vi "Read.vi"(8 "error in (no error)":errorcluster, 11 "Modbus_AI in":refnum<class "Modbus_AI.lvclass">) -> (0 "error out":errorcluster, 2 "Data Out":dbl, 3 "Modbus_AI out":refnum<class "Modbus_AI.lvclass">)   [LabVIEW 2021, in "Modbus_AI.lvclass"]
uses:
  Modbus_AI.lvclass
  Modbus_AI.lvclass/Modbus_AI.ctl
  Modbus_Master/Modbus_Master.lvclass
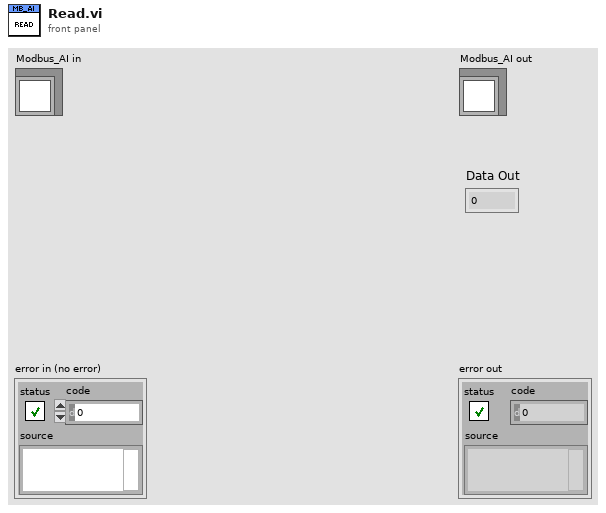
[diagram p1: front panel]
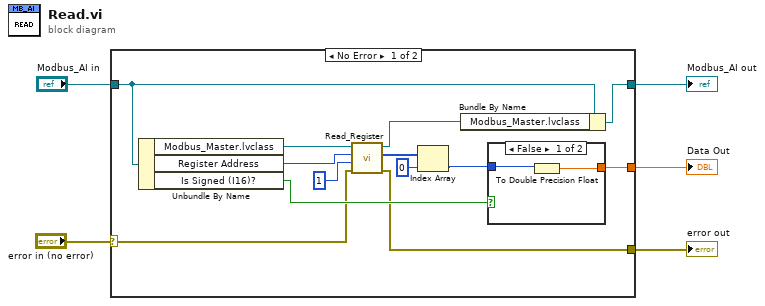
[diagram p0: block diagram]
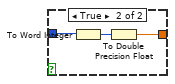
[diagram p2: hidden frame]
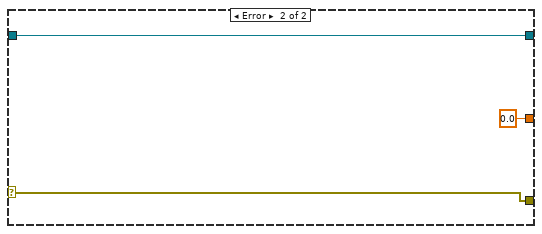
[diagram p3: hidden frame]
diagram:
  n1 = case shown="No Error" "error in (no error)" {
    selector: "error in (no error)" -> [w10 w25]
    tunnel: "Modbus_AI in" -> [w8 w24]
    tunnel: [w11 0.0] -> w3
    tunnel: [w9 w25] -> w2
    tunnel: [w7 w24] -> w1
    frame No Error {
      n2 = Unbundle By Name(w8) -> ("Modbus_Master.lvclass"=w18:refnum<class "Modbus_Master.lvclass">, "Register Address"=w17:u16, "Is Signed (I16)?"=w13:bool)
      n3 = call "Read_Register.vi"("error in (no error)"=w10, "Quantity"=u16 1, "Start Address"=w17, "Modbus_Master in"=w18) -> ("error out"=w9:errorcluster, "register values"=w15:u16[], "Modbus_Master out"=w6:refnum<class "Modbus_Master.lvclass">)  [unwired: 5 in]
      n4 = Index Array(array=w15, index=0) -> (element=w12:u16)
      n5 = Bundle By Name(cluster=w8, "Modbus_Master.lvclass"=w6) -> (w7:refnum<class "Modbus_AI.lvclass">)
      n6 = case shown="False" w13 {
        tunnel: w12 -> [w20 w23]
        tunnel: [w19 w21] -> w11
        frame False {
          n7 = To Double Precision Float(number=w20) -> (double precision float=w19:dbl)
        }
        frame True {
          n8 = To Word Integer(number=w23) -> (16bit integer=w22:i16)
          n9 = To Double Precision Float(number=w22) -> (double precision float=w21:dbl)
        }
      }
    }
    frame Error {
    }
  }
  "error out" <- w2
  "Modbus_AI out" <- w1
  "Data Out" <- w3
